vi "Force Cleanup.vi"(8 "error in":errorcluster) -> (0 "error out":errorcluster, 3 "context":refnum<class "zmq_context.lvclass">)   [LabVIEW 2019, in "RemoteControl.ZMQ.lvlib" / "ZMQ.ContextManager.lvlib"]
uses:
  ZMQ.ContextManager.lvlib
  <vilib>/addons/zeromq/zmq_context.lvclass
  Typedefs/Action--enum.ctl
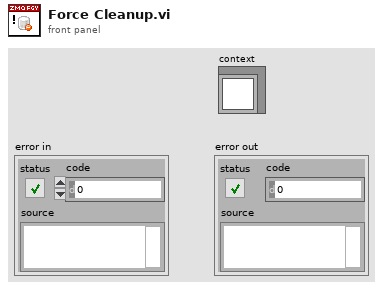
[diagram p1: front panel]
types:
  T1 = typedef "RemoteControl.ZMQ.lvlib/ZMQ.ContextManager.lvlib/Action--enum.ctl" = enum16{"Get Context", "Release Context", "Socket Opened", "Socket Closed", "Force Cleanup", "Set Context"}
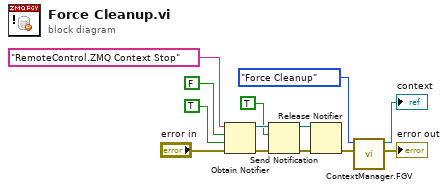
[diagram p0: block diagram]
diagram:
  n1 = Obtain Notifier(name (unnamed)="RemoteControl.ZMQ Context Stop", notification data type=FALSE, create if not found? (T)=TRUE, error in (no error)="error in") -> (notifier out=w7:refnum<notifier>, error out=w5:errorcluster)  [unwired: 1 out]
  n2 = Send Notification(notification=TRUE, notifier=w7, error in (no error)=w5) -> (notifier out=w4:refnum<notifier>, error out=w3:errorcluster)
  n3 = Release Notifier(notifier=w4, error in (no error)=w3) -> (error out=w1:errorcluster)  [unwired: 1 in, 2 out]
  n4 = call "ContextManager.FGV.vi"("error in"=w1, "action"=Action--enum."Force Cleanup") -> ("error out"=→"error out":errorcluster, "context out"=→"context":refnum<class "zmq_context.lvclass">)  [unwired: 8 in]
